vi "PID.vi"(6 "dt (s)":dbl=0.01 format="%#_13g", 8 "error in (no error)":errorcluster, 9 "PID gains":T1(array[cluster])=[{"proportional gain (Kc)"=1.0, "integral time (Ti, min)"=0.0, "derivative time (Td, min)"=0.0002}, {"proportional gain (Kc)"=1.0, "integral time (Ti, min)"=0.0, "derivative time (Td, min)"=0.0002}] {"derivative time (Td, min)" format="%.4f"; "integral time (Ti, min)" format="%.3f"; "proportional gain (Kc)" format="%.3f"}, 10 "目標":dbl[](array[numeric])=[0.0, 0.0] format="%#_13g", 11 "Reset":bool=TRUE) -> (0 "error out":errorcluster, 1 "ENC":dbl[](array[numeric])=[-6804.0, 6797.0], 2 "output":dbl[](array[numeric])=[100.0, -100.0], 3 "誤差":dbl[](array[numeric])=[6804.0, -6797.0], 5 "Waveform Graph":dbl[](graph)=[100.0, -100.0])   [LabVIEW 2019]
uses:
  <vilib>/addons/control/pid/pid.llb/PID (DBL Array).vi
  <vilib>/addons/control/pid/NI_PID_pid.lvlib
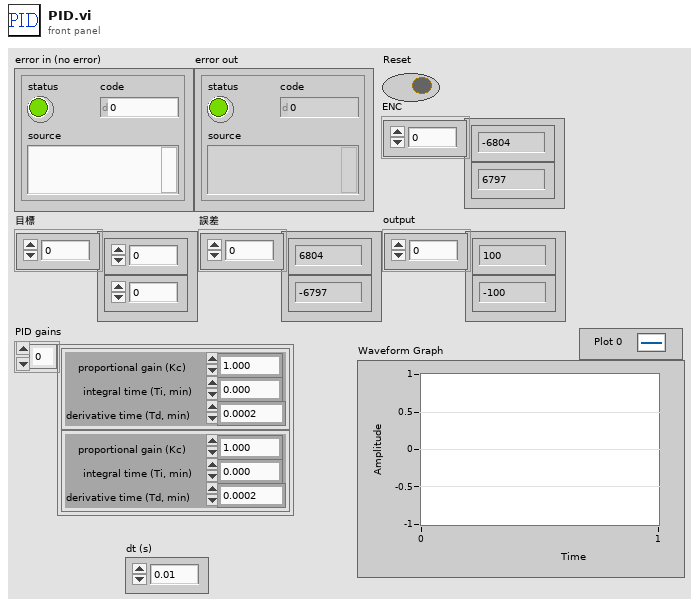
[diagram p1: front panel]
types:
  T1 = cluster{"proportional gain (Kc)":dbl, "integral time (Ti, min)":dbl, "derivative time (Td, min)":dbl}[]
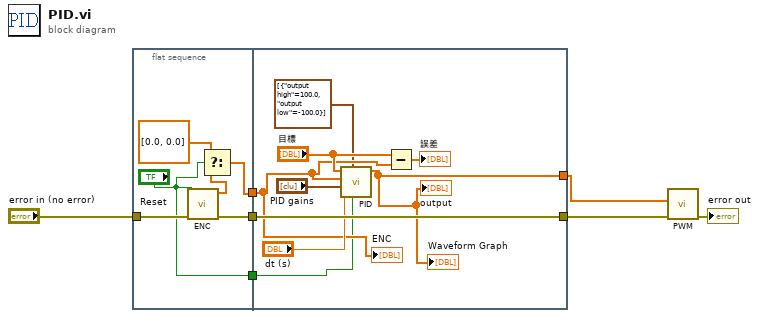
[diagram p0: block diagram]
diagram:
  n1 = flat-sequence {
    tunnel: "error in (no error)" -> [w13]
    tunnel: [w12] -> w5
    tunnel: [w11] -> w4
    tunnel: ["Reset"] -> w1
    tunnel: [w22] -> w2
    tunnel: w5 -> [w22]
    tunnel: w4 -> [w17]
    tunnel: [w15] -> w3
    tunnel: w1 -> [w14]
    frame #0 {
      n2 = call "ENC.vi"("error in (no error)"=w13, "Reset"="Reset") -> ("error out"=w12:errorcluster, "ENC"=w10:dbl[])  [unwired: 6 in, 2 out]
      n3 = Select(t=dbl[] [0.0, 0.0], s="Reset", f=w10) -> (s? t:f=w11:dbl[])
    }
    frame #1 {
      n4 = call-poly <vilib>:"PID.vi"("reinitialize? (F)"=w14, "output range"=cluster{"output high":dbl, "output low":dbl}[] [{"output high"=100.0, "output low"=-100.0}], "dt (s)"="dt (s)", "PID gains"="PID gains", "process variable"=w17, "setpoint"="目標") -> ("output"=w15:dbl[])  [unwired: 4 in, 1 out]
      "output" <- w15
      "Waveform Graph" <- w15
      n5 = Subtract(x="目標", y=w17) -> (x-y=→"誤差":dbl[])
      "ENC" <- w17
    }
  }
  n6 = call "PWM.vi"("error in (no error)"=w2, "power"=w3) -> ("error out"=→"error out":errorcluster)  [unwired: 9 in]
